vi "subReplaceSourceLibaryWithBuiltLib.vi"(8 "error in (no error)":errorcluster, 10 "ProjectItem in":refnum<class "ProjectItem.lvclass">, 11 "BuildManager in":refnum<class "BuildManager.lvclass">) -> (0 "error out":errorcluster, 3 "BuildManager out":refnum<class "BuildManager.lvclass">)   [LabVIEW 2019, in "SolutionBuilder.lvlib" / "BuildManager.lvclass"]
uses:
  BuildManager.lvclass
  ProjectItem/ProjectItem.lvclass
  ProjectItem/ProjectItem.lvclass/ProjectItem.ctl
  LogInfo.ctl
  BuildManager.lvclass/BuildManager.ctl
  SolutionBuilder.lvlib
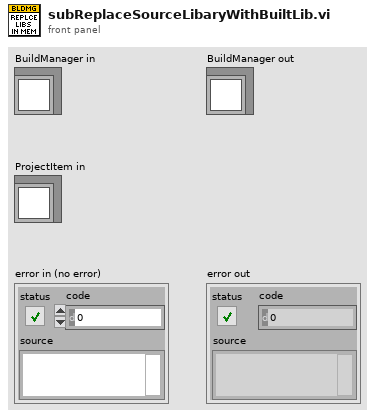
[diagram p1: front panel]
types:
  T1 = typedef "SolutionBuilder.lvlib/BuildManager.lvclass/LogInfo.ctl" = cluster{"Build spec name":string, "Source path":path, "Destination path":path, "Target":string}
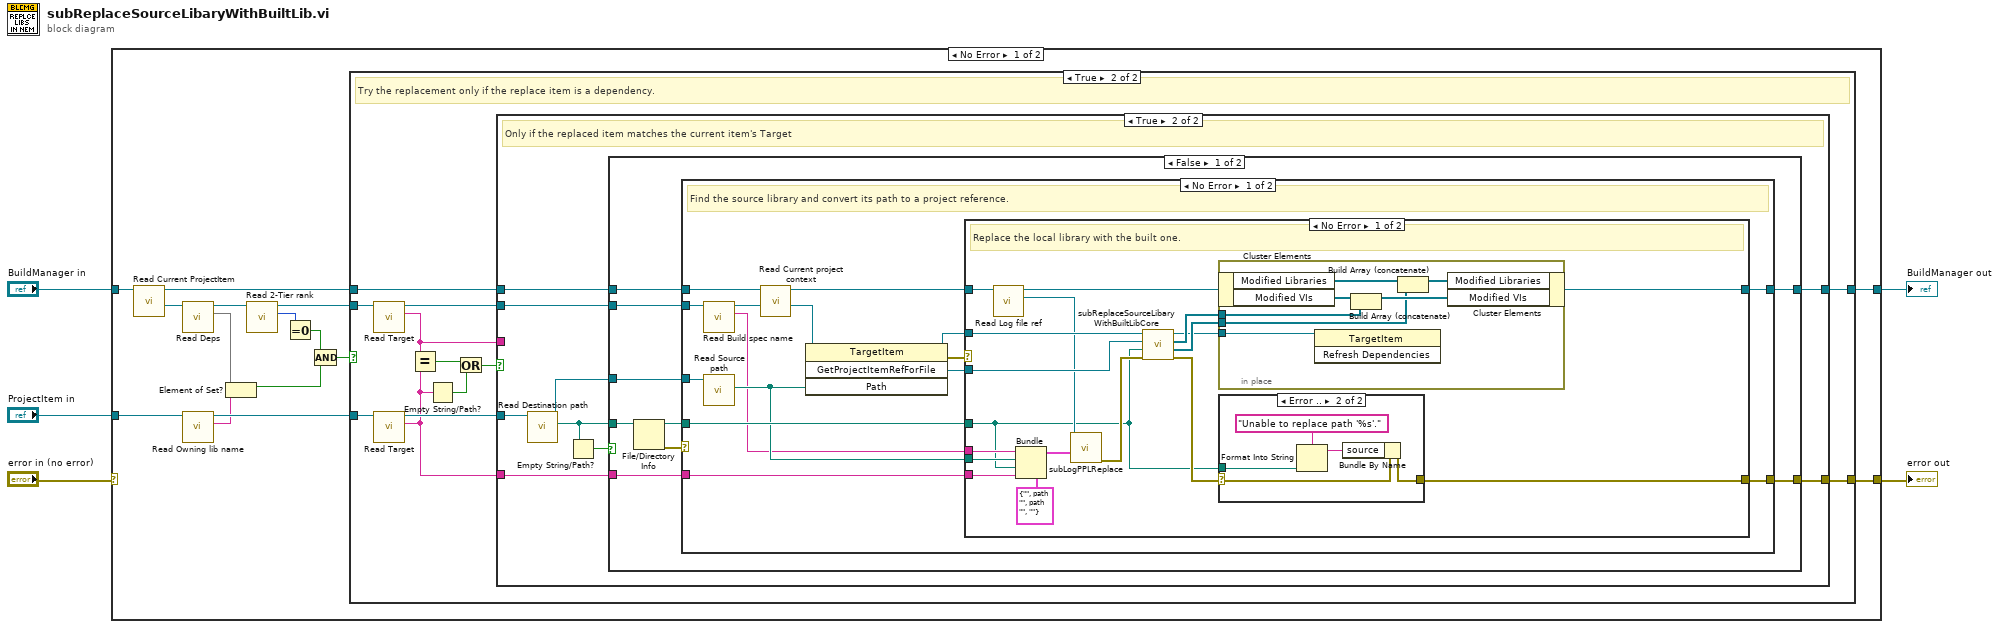
[diagram p0: block diagram]
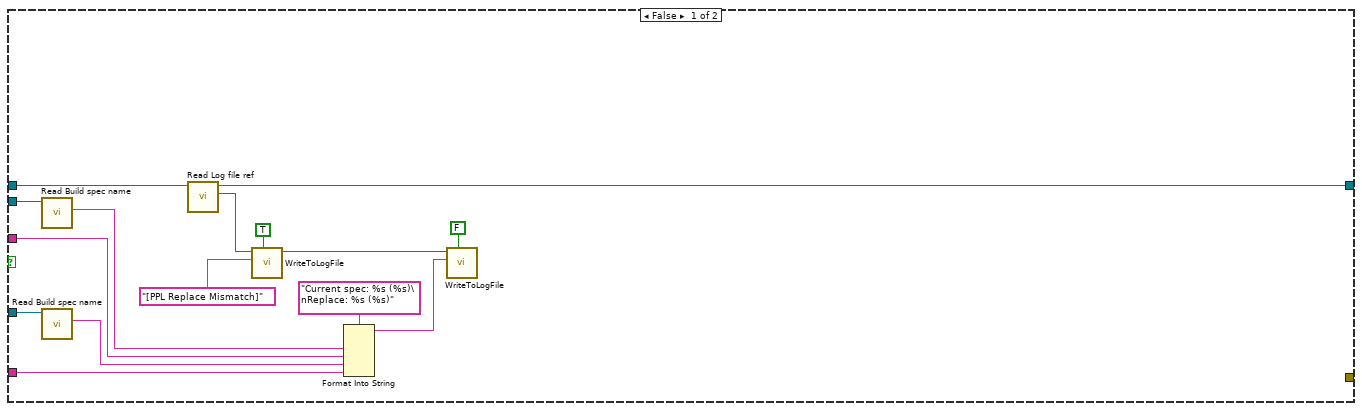
[diagram p3: hidden frame]
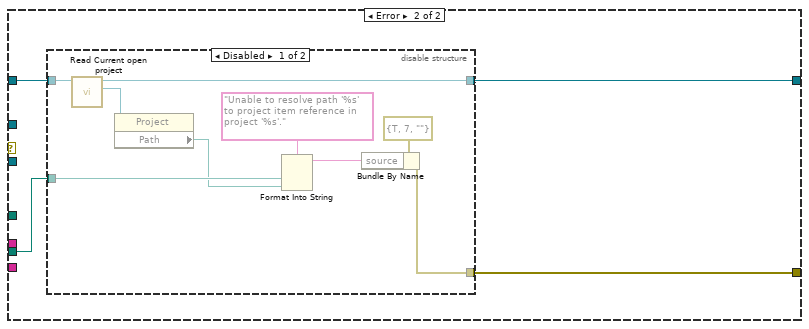
[diagram p5: hidden frame]
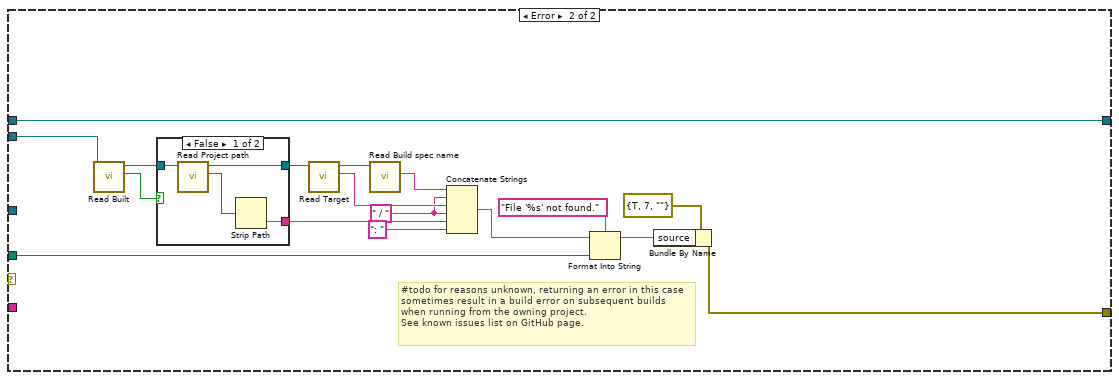
[diagram p7: hidden frame]
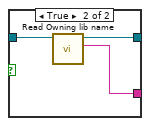
[diagram p8: hidden frame]
diagram:
  n1 = case shown="No Error" "error in (no error)" {
    selector: "error in (no error)" -> [_ w153]
    tunnel: [w20 w152] -> w5
    tunnel: "BuildManager in" -> [w17 w152]
    tunnel: "ProjectItem in" -> [w15 _]
    tunnel: [w19 w153] -> w1
    frame No Error {
      n2 = call "Read Current ProjectItem.vi"("BuildManager in"=w17) -> ("Current ProjectItem"=w16:refnum<class "ProjectItem.lvclass">, "BuildManager out"=w18:refnum<class "BuildManager.lvclass">)  [unwired: 7 in, 2 out]
      n3 = call "Read Deps.vi"("ProjectItem in"=w16) -> ("Deps"=w13:set{string}, "ProjectItem out"=w11:refnum<class "ProjectItem.lvclass">)  [unwired: 9 in]
      n4 = call "Read Owning lib name.vi"("ProjectItem in"=w15) -> ("Owning lib name"=w12:string, "ProjectItem out"=w14:refnum<class "ProjectItem.lvclass">)  [unwired: 9 in]
      n5 = Element of Set?(10:w12, 11:w13) -> (3:w8:bool)
      n6 = call "Read 2-Tier rank.vi"("ProjectItem in"=w11) -> ("2-Tier rank"=w10:u8, "ProjectItem out"=w6:refnum<class "ProjectItem.lvclass">)  [unwired: 9 in]
      n7 = Equal To 0?(x=w10) -> (x = 0?=w9:bool)
      n8 = Compound Arithmetic op=AND(w9, w8) -> (w7:bool)
      n9 = case shown="True" w7 {
        tunnel: [w21 w33] -> w20
        tunnel: [_ w32] -> w19
        tunnel: w18 -> [w21 w31]
        tunnel: w14 -> [_ w28]
        tunnel: w6 -> [_ w29]
        frame False {
        }
        frame True {
          # "Try the replacement only if the replace item is a dependency."
          n10 = call "Read Target.vi"("ProjectItem in"=w29) -> ("Target"=w22:string, "ProjectItem out"=w30:refnum<class "ProjectItem.lvclass">)  [unwired: 9 in]
          n11 = call "Read Target.vi"("ProjectItem in"=w28) -> ("Target"=w26:string, "ProjectItem out"=w27:refnum<class "ProjectItem.lvclass">)  [unwired: 9 in]
          n12 = Equal?(x=w22, y=w26) -> (x = y?=w25:bool)
          n13 = Empty String/Path?(string/path=w26) -> (empty?=w24:bool)
          n14 = Or(x=w25, y=w24) -> (x .or. y?=w23:bool)
          n15 = case shown="True" w23 {
            tunnel: [w46 w57] -> w33
            tunnel: [_ w53] -> w32
            tunnel: w31 -> [w45 w52]
            tunnel: w30 -> [w47 w51]
            tunnel: w27 -> [w48 w50]
            tunnel: w26 -> [w34 w49]
            tunnel: w22 -> [w36 _]
            frame False {
              n16 = call "Read Build spec name.vi"("ProjectItem in"=w47) -> ("Build spec name"=w37:string)  [unwired: 9 in, 1 out]
              n17 = call "Read Build spec name.vi"("ProjectItem in"=w48) -> ("Build spec name"=w35:string)  [unwired: 9 in, 1 out]
              n18 = call "Read Log file ref.vi"("BuildManager in"=w45) -> ("Log file ref"=w38:refnum<file>, "BuildManager out"=w46:refnum<class "BuildManager.lvclass">)  [unwired: 9 in]
              n19 = call "WriteToLogFile.vi"("Prepend timestamp"=TRUE, "Log entry"="[PPL Replace Mismatch]" ("format string"), "Byte Stream File in"=w38) -> ("refnum out"=w40:refnum<file>)  [unwired: 7 in, 1 out]
              n20 = Format Into String(format string="Current spec: %s (%s)\nReplace: %s (%s)", w37, w36, w35, w34) -> (resulting string=w39:string)  [unwired: 2 in, 1 out]
              n21 = call "WriteToLogFile.vi"("Prepend timestamp"=FALSE, "Log entry"=w39, "Byte Stream File in"=w40) -> ()  [unwired: 7 in, 2 out]
            }
            frame True {
              # "Only if the replaced item matches the current item's Target"
              n22 = call "Read Destination path.vi"("ProjectItem in"=w50) -> ("Destination path"=w55:path, "ProjectItem out"=w54:refnum<class "ProjectItem.lvclass">)  [unwired: 9 in]
              n23 = Empty String/Path?(string/path=w55) -> (empty?=w56:bool)
              n24 = case shown="False" w56 {
                tunnel: w54 -> [w66 _]
                tunnel: w55 -> [w62 _]
                tunnel: w52 -> [w64 w151]
                tunnel: [w65 w151] -> w57
                tunnel: [w60 _] -> w53
                tunnel: w51 -> [w59 _]
                tunnel: w49 -> [w58 _]
                frame False {
                  n25 = File/Directory Info(path=w62) -> (path out=w63:path, error out=w61:errorcluster)  [unwired: 1 in, 5 out]
                  n26 = case shown="No Error" w61 {
                    tunnel: w66 -> [w80 _]
                    tunnel: [w78 w143] -> w65
                    tunnel: w64 -> [w76 w143]
                    tunnel: w63 -> [w73 w139]
                    tunnel: [w71 w138] -> w60
                    tunnel: w59 -> [w70 w133]
                    tunnel: w58 -> [w67 _]
                    frame No Error {
                      # "Find the source library and convert its path to a project reference."
                      n27 = call "Read Build spec name.vi"("ProjectItem in"=w70) -> ("Build spec name"=w68:string, "ProjectItem out"=w69:refnum<class "ProjectItem.lvclass">)  [unwired: 9 in]
                      n28 = call "Read Source path.vi"("ProjectItem in"=w80) -> ("Source path"=w72:path)  [unwired: 9 in, 1 out]
                      n29 = call "Read Current project context.vi"("Current ProjectItem"=w69, "BuildManager in"=w76) -> ("Project context"=w74:refnum<vi>, "BuildManager out"=w75:refnum<class "BuildManager.lvclass">)  [unwired: 8 in]
                      n30 = invoke class="TargetItem" method="GetProjectItemRefForFile"(reference=w74, "Path"=w72) -> (reference out=w77:refnum<vi>, error out=w79:errorcluster, "GetProjectItemRefForFile"=w81:refnum<vi>)  [unwired: 2 in, 1 out]
                      n31 = case shown="No Error" w79 {
                        tunnel: w81 -> [w99 _]
                        tunnel: w73 -> [w83 _]
                        tunnel: w75 -> [w91 w113]
                        tunnel: [w96 w114] -> w78
                        tunnel: w77 -> [w92 _]
                        tunnel: w72 -> [w84 w116]
                        tunnel: [w95 w115] -> w71
                        tunnel: w68 -> [w85 _]
                        tunnel: w67 -> [w82 _]
                        frame No Error {
                          # "Replace the local library with the built one."
                          n32 = call "Read Log file ref.vi"("BuildManager in"=w91) -> ("Log file ref"=w88:refnum<file>, "BuildManager out"=w90:refnum<class "BuildManager.lvclass">)  [unwired: 9 in]
                          n33 = Bundle(cluster=T1 {"Build spec name"="", "Source path"=path "", "Destination path"=path "", "Target"=""} ("Log info"), "Build spec name"=w85, "Source path"=w84, "Destination path"=w83, "Target"=w82) -> (w86:T1)
                          n34 = call "subLogPPLReplace.vi"("Log info"=w86, "Byte Stream File in"=w88) -> ("error out"=w89:errorcluster)  [unwired: 8 in, 1 out]
                          n35 = call "subReplaceSourceLibaryWithBuiltLibCore.vi"("error in (no error)"=w89, "path in"=w83, "GetProjectItemRefForFile"=w99, "TargetItem in"=w92) -> ("error out"=w94:errorcluster, "Modified Libraries"=w97:refnum<vi>[], "Modified VIs"=w98:refnum<vi>[], "TargetItem out"=w93:refnum<vi>)  [unwired: 4 in]
                          n36 = in-place {
                            in-place-border: w98 -> [w111]
                            in-place-border: w97 -> [w108]
                            in-place-border: w93 -> [w106]
                            n37 = in-place-cluster #1(w90) -> ("Modified Libraries"=w109:refnum<vi>[], "Modified VIs"=w112:refnum<vi>[])
                            n38 = invoke class="TargetItem" method="Refresh Dependencies"(reference=w106) -> ()  [unwired: 2 in, 3 out]
                            n39 = Build Array (concatenate)(w112, w111) -> (w110:refnum<vi>[])
                            n40 = Build Array (concatenate)(w109, w108) -> (w107:refnum<vi>[])
                            n41 = in-place-cluster #1("Modified Libraries"=w107, "Modified VIs"=w110) -> (w96:refnum<class "BuildManager.lvclass">)
                          }
                          n42 = case shown="Error .." w94 {
                            selector: w94 -> [w100 w101]
                            tunnel: [w100 w105] -> w95
                            tunnel: w83 -> [_ w103]
                            frame No Error {
                            }
                            frame Error {
                              n43 = Format Into String(format string="Unable to replace path '%s'.", w103) -> (resulting string=w102:string)  [unwired: 2 in, 1 out]
                              n44 = Bundle By Name(cluster=w101, "source"=w102) -> (w105:errorcluster)
                            }
                          }
                        }
                        frame Error {
                          n45 = disable-structure shown="Disabled" {
                            disable-tunnel: w116 -> [w122 _]
                            disable-tunnel: [w121 _] -> w115
                            disable-tunnel: [w120 w126] -> w114
                            disable-tunnel: w113 -> [w119 w126]
                            frame Disabled {
                              n46 = call "Read Current open project.vi"("BuildManager in"=w119) -> ("Current open project"=w118:refnum<vi>, "BuildManager out"=w120:refnum<class "BuildManager.lvclass">)  [unwired: 9 in]
                              n47 = property class="Project"(reference=w118) -> ("Path"=w117:path)  [unwired: 1 in, 2 out]
                              n48 = Format Into String(format string="Unable to resolve path '%s' to project item reference in project '%s'.", w122, w117) -> (resulting string=w123:string)  [unwired: 2 in, 1 out]
                              n49 = Bundle By Name(cluster=errorcluster {"status"=TRUE, "code"=7, "source"=""} ("error out"), "source"=w123) -> (w121:errorcluster)
                            }
                            frame Enabled {
                            }
                          }
                        }
                      }
                    }
                    frame Error {
                      w130 = " / " ("string")
                      # "#todo for reasons unknown, returning an error in this case sometimes result in a build error on subsequent builds when running from the owning project.\nSee known issues list on GitHub page."
                      n50 = call "Read Built.vi"("ProjectItem in"=w133) -> ("Built"=w135:bool, "ProjectItem out"=w136:refnum<class "ProjectItem.lvclass">)  [unwired: 9 in]
                      n51 = case shown="False" w135 {
                        tunnel: w136 -> [w147 w150]
                        tunnel: [w145 w148] -> w129
                        tunnel: [w144 w149] -> w134
                        frame False {
                          n52 = call "Read Project path.vi"("ProjectItem in"=w147) -> ("Project path"=w146:path, "ProjectItem out"=w144:refnum<class "ProjectItem.lvclass">)  [unwired: 9 in]
                          n53 = Strip Path(path=w146) -> (name=w145:string)  [unwired: 1 out]
                        }
                        frame True {
                          n54 = call "Read Owning lib name.vi"("ProjectItem in"=w150) -> ("Owning lib name"=w148:string, "ProjectItem out"=w149:refnum<class "ProjectItem.lvclass">)  [unwired: 9 in]
                        }
                      }
                      n55 = call "Read Target.vi"("ProjectItem in"=w134) -> ("Target"=w131:string, "ProjectItem out"=w137:refnum<class "ProjectItem.lvclass">)  [unwired: 9 in]
                      n56 = call "Read Build spec name.vi"("ProjectItem in"=w137) -> ("Build spec name"=w132:string)  [unwired: 9 in, 1 out]
                      n57 = Concatenate Strings(w132, w130, w131, w130, w129, ": " ("string")) -> (w127:string)
                      n58 = Format Into String(format string="File '%s' not found.", initial string=w127, w139) -> (resulting string=w140:string)  [unwired: 1 in, 1 out]
                      n59 = Bundle By Name(cluster=errorcluster {"status"=TRUE, "code"=7, "source"=""} ("error out"), "source"=w140) -> (w138:errorcluster)
                    }
                  }
                }
                frame True {
                }
              }
            }
          }
        }
      }
    }
    frame Error {
    }
  }
  "BuildManager out" <- w5
  "error out" <- w1
